vi "PicoScope6000GetTriggerInfo.vi"(0 "handle in":i16, 5 "Rapid Block Acquisition Settings":T1={"preTriggerSamples"=0, "postTriggerSamples"=1000, "timebase"=10, "Four Channel Device"=TRUE, "Oversample"=1, "Number of Captures"=8}, 9 "Sample Rate":sgl, 11 "error in":errorcluster) -> (4 "handle out":i16, 6 "Trigger Info":T2(array[cluster]), 10 "Trigger Offsets":cluster{u64, sgl}[](array[cluster]) {"?" format="%#_5p"}, 15 "error out":errorcluster)   [LabVIEW 2016]
doc: "This VI gets trigger timestamped data using rapid block mode. It outputs one-dimensional array for each memory segment."
uses:
  ps6000.dll
panel:
  out "Number of Captures":u32=1
  in  "fromSegmentIndex":u32
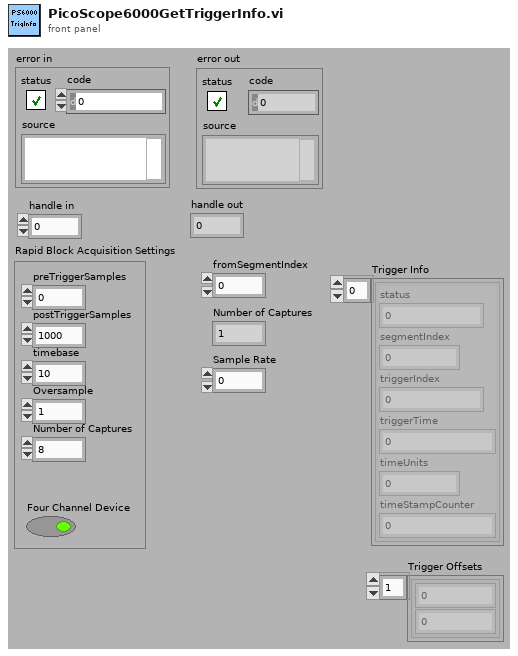
[diagram p1: front panel]
types:
  T1 = cluster{"preTriggerSamples":u32, "postTriggerSamples":u32, "timebase":u32, "Four Channel Device":bool, "Oversample":i16, "Number of Captures":u32}
  T2 = cluster{"status":u32, "segmentIndex":u32, "triggerIndex":u32, "triggerTime":i64, "timeUnits":i16, "timeStampCounter":u64}[]
  T3 = cluster{"status":u32, "segmentIndex":u32, "triggerIndex":u32, "triggerTime":i64, "timeUnits":i16, "reserved0":i16, "timeStampCounter":u64}
  T4 = cluster{"status":u32, "segmentIndex":u32, "triggerIndex":u32, "triggerTime":i64, "timeUnits":i16, "timeStampCounter":u64}
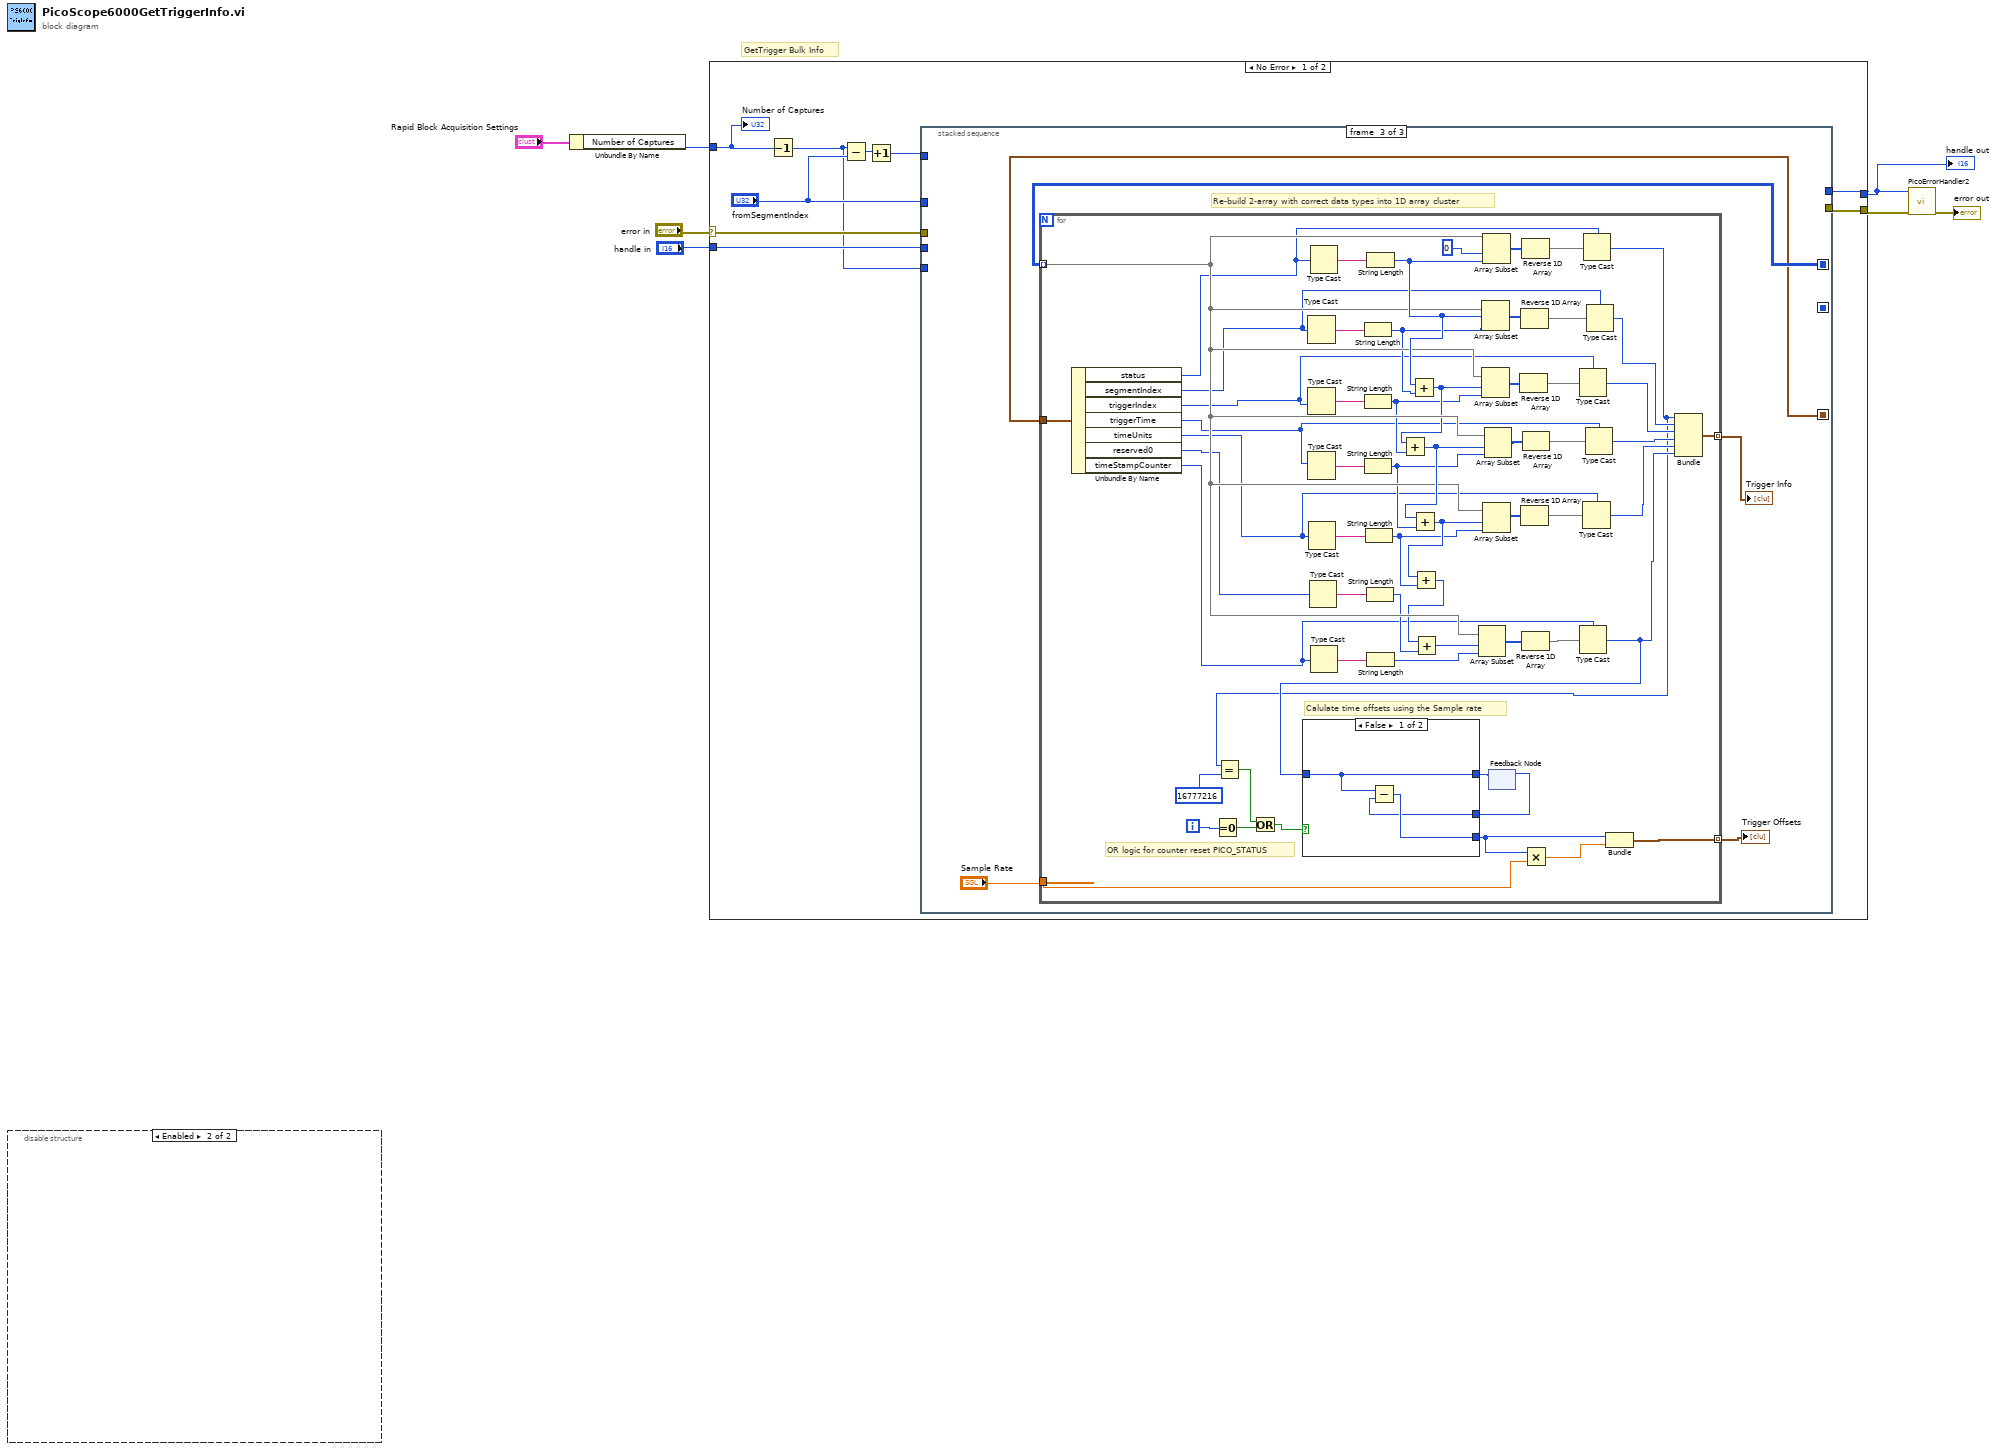
[diagram p0: block diagram]
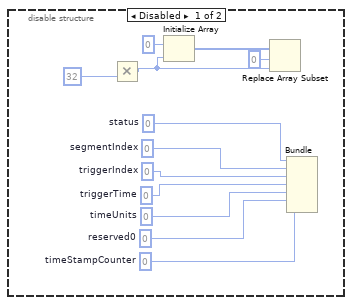
[diagram p2: hidden frame]
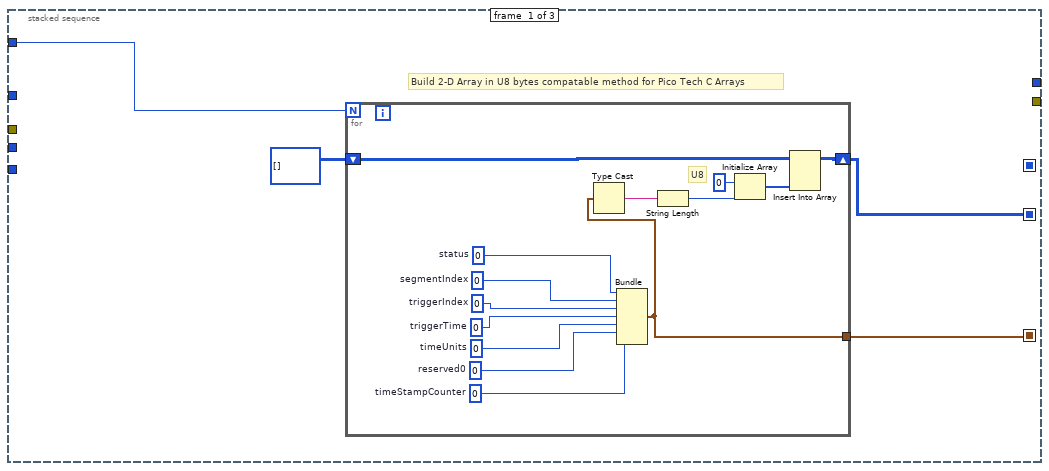
[diagram p3: hidden frame]
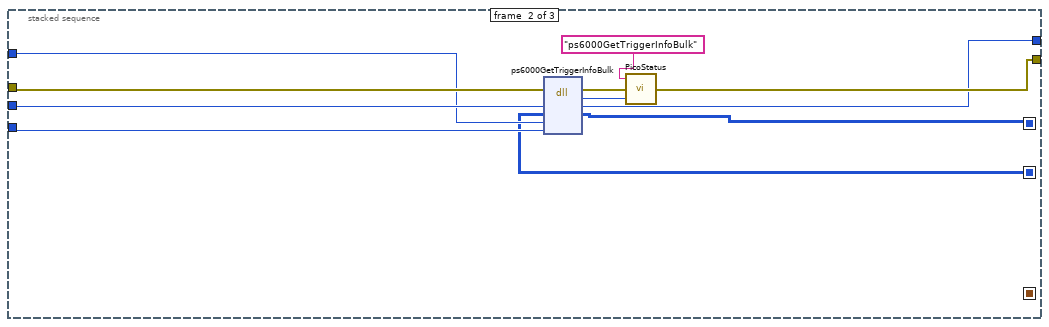
[diagram p4: hidden frame]
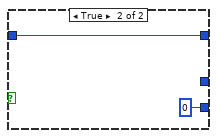
[diagram p5: hidden frame]
diagram:
  # "GetTrigger Bulk Info"
  n1 = disable-structure shown="Enabled" {
    frame Disabled {
      w15 = u64 0  # timeStampCounter
      w13 = i16 0  # reserved0
      w14 = i16 0  # timeUnits
      w16 = i64 0  # triggerTime
      w17 = u32 0  # triggerIndex
      w18 = u32 0  # segmentIndex
      w19 = u32 0  # status
      n2 = Multiply(y=u32 32) -> (x*y=w11:u32)  [unwired: 1 in]
      n3 = Initialize Array(u8 0 ("element"), w11) -> (w12:u8[])
      n4 = Replace Array Subset(array=w12, new element=w11, index=0) -> ()  [unwired: 1 out]
      n5 = Bundle("status"=w19, "segmentIndex"=w18, "triggerIndex"=w17, "triggerTime"=w16, "timeUnits"=w14, "reserved0"=w13, "timeStampCounter"=w15) -> ()  [unwired: 1 in, 1 out]
    }
    frame Enabled {
    }
  }
  n6 = Unbundle By Name("Rapid Block Acquisition Settings") -> ("Number of Captures"=w5:u32)
  n7 = case shown="No Error" "error in" {
    selector: "error in" -> [w27 w129]
    tunnel: [w23 w129] -> w3
    tunnel: "handle in" -> [w26 w128]
    tunnel: [w22 w128] -> w4
    tunnel: w5 -> [w28 _]
    frame No Error {
      n8 = Decrement(x=w28) -> (x-1=w24:u32)
      n9 = Subtract(x=w24, y="fromSegmentIndex") -> (x-y=w21:u32)
      n10 = Increment(x=w21) -> (x+1=w20:u32)
      n11 = stacked-sequence {
        seq-local: [w30 _ _] -> [_ w50 _]
        seq-local: [w29 _ _] -> [_ w48 _]
        seq-local: [_ w49 _] -> [_ _ w63]
        seq-local: [_ w48 _] -> [_ _ w59]
        tunnel: w20 -> [w32 _ _]
        tunnel: w27 -> [_ w55 _]
        tunnel: w26 -> [_ w53 _]
        tunnel: "fromSegmentIndex" -> [_ w52 _]
        tunnel: w24 -> [_ w51 _]
        tunnel: [_ w54 _] -> w23
        tunnel: [_ w47 _] -> w22
        frame #0 {
          # "Build 2-D Array in U8 bytes compatable method for Pico Tech C Arrays"
          n12 = for {
            N: w32 -> [_]
            shift-right: [w34] -> w30
            shift-left: u8[][] [] -> [w35]
            tunnel: [w33] -> w29
            w42 = u64 0  # timeStampCounter
            w40 = i16 0  # reserved0
            w41 = i16 0  # timeUnits
            w43 = i64 0  # triggerTime
            w44 = u32 0  # triggerIndex
            w45 = u32 0  # segmentIndex
            w46 = u32 0  # status
            # "U8"
            n13 = Bundle("status"=w46, "segmentIndex"=w45, "triggerIndex"=w44, "triggerTime"=w43, "timeUnits"=w41, "reserved0"=w40, "timeStampCounter"=w42) -> (w33:T3)  [unwired: 1 in]
            n14 = Type Cast(x=w33) -> (*(type *) &x=w39:string)  [unwired: 1 in]
            n15 = String Length(string=w39) -> (length=w37:i32)
            n16 = Initialize Array(u8 0 ("element"), w37) -> (w36:u8[])
            n17 = Insert Into Array(array=w35, new element=w36) -> (w34:u8[][])  [unwired: 2 in]
          }
        }
        frame #1 {
          n18 = dll-call lib="ps6000.dll" fn="ps6000GetTriggerInfoBulk" ("ps3000.dll:_ps3000_open_unit@0")(error in=w55, "handle"=w53, "triggerInfo"=w50, "fromSegmentIndex"=w52, "toSegmentIndex"=w51) -> (error out=w58:errorcluster, "PICO_STATUS"=w57:u32, "handle"=w47:i16, "triggerInfo"=w49:u8[][])  [unwired: 4 in, 1 out]
          n19 = call "PicoStatus.vi"("PICO STATUS"=w57, "error in"=w58, "source"="ps6000GetTriggerInfoBulk") -> ("error out"=w54:errorcluster)
        }
        frame #2 {
          # "Re-build 2-array with correct data types into 1D array cluster"
          n20 = for {
            tunnel: w63 -> [w84] mode=indexing
            tunnel: [w119] -> w62 mode=indexing
            tunnel: [w102] -> w61 mode=indexing
            tunnel: "Sample Rate" -> [w101]
            tunnel: w59 -> [w71]
            i -> [w105]
            # "Calulate time offsets using the Sample rate"
            # "OR logic for counter reset PICO_STATUS"
            n21 = Unbundle By Name(w71) -> ("status"=w70:u32, "segmentIndex"=w69:u32, "triggerIndex"=w64:u32, "triggerTime"=w65:i64, "timeUnits"=w66:i16, "reserved0"=w67:i16, "timeStampCounter"=w68:u64)
            n22 = Equal To 0?(x=w105) -> (x = 0?=w76:bool)
            n23 = Type Cast(x=w69) -> (*(type *) &x=w97:string)  [unwired: 1 in]
            n24 = Type Cast(x=w64) -> (*(type *) &x=w96:string)  [unwired: 1 in]
            n25 = Type Cast(x=w65) -> (*(type *) &x=w95:string)  [unwired: 1 in]
            n26 = Type Cast(x=w66) -> (*(type *) &x=w94:string)  [unwired: 1 in]
            n27 = Type Cast(x=w67) -> (*(type *) &x=w93:string)  [unwired: 1 in]
            n28 = Type Cast(x=w70) -> (*(type *) &x=w98:string)  [unwired: 1 in]
            n29 = Type Cast(x=w68) -> (*(type *) &x=w88:string)  [unwired: 1 in]
            n30 = String Length(string=w97) -> (length=w82:i32)
            n31 = String Length(string=w96) -> (length=w80:i32)
            n32 = String Length(string=w95) -> (length=w79:i32)
            n33 = String Length(string=w94) -> (length=w78:i32)
            n34 = String Length(string=w93) -> (length=w77:i32)
            n35 = String Length(string=w98) -> (length=w89:i32)
            n36 = String Length(string=w88) -> (length=w86:i32)
            n37 = Add(x=w89, y=w82) -> (x+y=w81:i32)
            n38 = Add(x=w81, y=w80) -> (x+y=w92:i32)
            n39 = Add(x=w92, y=w79) -> (x+y=w91:i32)
            n40 = Add(x=w91, y=w78) -> (x+y=w83:i32)
            n41 = Add(x=w83, y=w77) -> (x+y=w87:i32)
            n42 = Array Subset(array=w84, index=w87, length=w86) -> (w85:u8[])
            n43 = Array Subset(array=w84, index=w89, length=w82) -> (w118:u8[])
            n44 = Array Subset(array=w84, index=w81, length=w80) -> (w113:u8[])
            n45 = Array Subset(array=w84, index=0, length=w89) -> (w116:u8[])
            n46 = Array Subset(array=w84, index=w91, length=w78) -> (w110:u8[])
            n47 = Array Subset(array=w84, index=w92, length=w79) -> (w112:u8[])
            n48 = feedback #1() -> (w103:u64)  [unwired: 1 in]
            n49 = Reverse 1D Array(array=w113) -> (reversed array=w114:u8[])
            n50 = Reverse 1D Array(array=w118) -> (reversed array=w117:u8[])
            n51 = Reverse 1D Array(array=w110) -> (reversed array=w109:u8[])
            n52 = Reverse 1D Array(array=w116) -> (reversed array=w115:u8[])
            n53 = Reverse 1D Array(array=w85) -> (reversed array=w108:u8[])
            n54 = Reverse 1D Array(array=w112) -> (reversed array=w111:u8[])
            n55 = Type Cast(type=w64, x=w114) -> (*(type *) &x=w122:u32)
            n56 = Type Cast(type=w68, x=w108) -> (*(type *) &x=w106:u64)
            n57 = Type Cast(type=w66, x=w109) -> (*(type *) &x=w120:i16)
            n58 = Type Cast(type=w70, x=w115) -> (*(type *) &x=w72:u32)
            n59 = Equal?(x=w72, y=u32 16777216 ("status")) -> (x = y?=w74:bool)
            n60 = Or(x=w74, y=w76) -> (x .or. y?=w75:bool)
            n61 = case shown="False" w75 {
              tunnel: w106 -> [w124 w127]
              tunnel: [w124 w127] -> w104
              tunnel: w103 -> [w123 _]
              tunnel: [w125 u64 0] -> w100
              frame False {
                n62 = Subtract(x=w124, y=w123) -> (x-y=w125:u64)
              }
              frame True {
              }
            }
            n63 = feedback-in #1(w104) -> ()
            n64 = Multiply(x=w100, y=w101) -> (x*y=w99:sgl)
            n65 = Type Cast(type=w65, x=w111) -> (*(type *) &x=w121:i64)
            n66 = Type Cast(type=w69, x=w117) -> (*(type *) &x=w107:u32)
            n67 = Bundle(w100, w99) -> (w102:cluster{u64, sgl})  [unwired: 1 in]
            n68 = Bundle("status"=w72, "segmentIndex"=w107, "triggerIndex"=w122, "triggerTime"=w121, "timeUnits"=w120, "timeStampCounter"=w106) -> (w119:T4)  [unwired: 1 in]
          }
          "Trigger Info" <- w62
          "Trigger Offsets" <- w61
        }
      }
      "Number of Captures" <- w28
    }
    frame Error {
    }
  }
  "handle out" <- w4
  n69 = call "PicoErrorHandler2.vi"("error in (no error)"=w3, "handle In"=w4) -> ("error out"=→"error out":errorcluster)  [unwired: 9 in]
